vi "UnscentedKalmanFilter_SetXHat_Single.vi"(9 "xHat Value":dbl, 10 "Row":i32, 11 "in UnscentedKalmanFiilter":T1) -> (0 "Error":bool, 3 "out UnscentedKalmanFiilter":T1)   [LabVIEW 2019, in "Trajectory_Library.lvlib"]
doc: "Set an element of the initial state estimate x-hat.\n \nInputs:\n - inUnscentedKalmanFilter -- filter data cluster\n - row -- Row of x-hat.\n - value -- Value for element of x-hat.\n\nOutputs:\n - outUnscentedKalmanFilter -- updated filter data cluster\n - error -- If TRUE, an error occured."
uses:
  Trajectory_Library.lvlib
  <vilib>/Analysis/Matrix/Datatypes/RealMatrix.ctl
  <vilib>/Analysis/Matrix/NI_Matrix.lvlib
  TypeDef/MERWE_SCALED_SIGMA_PTS.ctl
  TypeDef/UNSCENTED_KALMAN_FILTER.ctl
  TypeDef/CALLBACK_FUNC_TYPE.ctl
panel:
  # "State Estimate <Statess,1>"
  # "<States, States>"
  # "<States, ?>"
  # "<Statess,  States>"
  # "<Outputs, Outputs>"
  # "<?, 1>"
  # "<?, 1>"
  # "State Estimate <Statess,1>"
  # "<States, States>"
  # "<States, ?>"
  # "<Statess,  States>"
  # "<Outputs, Outputs>"
  # "<?, 1>"
  # "<?, 1>"
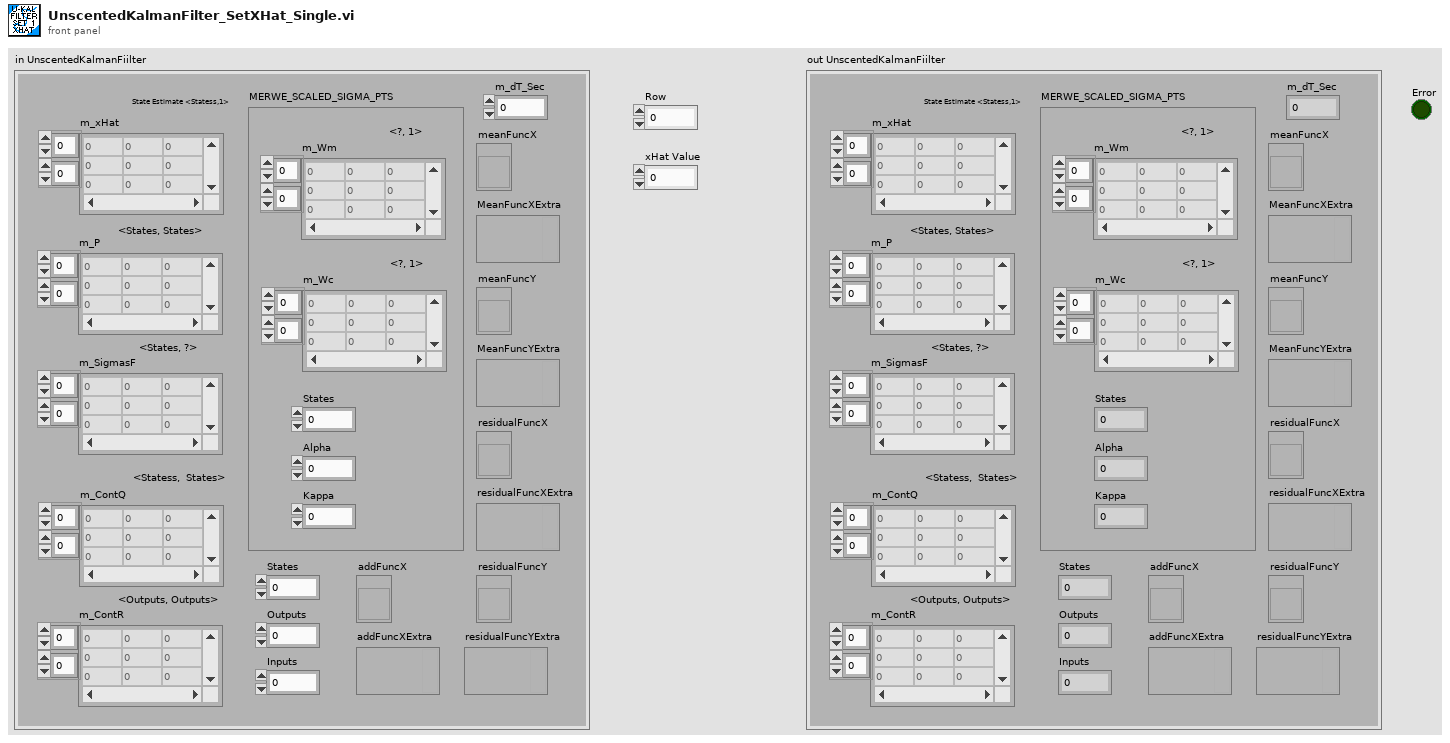
[diagram p1: front panel]
types:
  T1 = typedef "Trajectory_Library.lvlib/UNSCENTED_KALMAN_FILTER.ctl" = cluster{"m_P":T2, "m_xHat":T2, "States":i32, "Outputs":i32, "m_ContR":T2, "m_ContQ":T2, "m_SigmasF":T2, "m_dT_Sec":dbl, "MERWE_SCALED_SIGMA_PTS":T3, "meanFuncX":T4, "meanFuncY":T4, "residualFuncX":T4, "residualFuncY":T4, "addFuncX":T4, "addFuncXExtra":variant, "residualFuncYExtra":variant, "residualFuncXExtra":variant, "MeanFuncYExtra":variant, "MeanFuncXExtra":variant, "Inputs":i32}
  T2 = typedef "NI_Matrix.lvlib/RealMatrix.ctl" = dbl[][]
  T3 = typedef "Trajectory_Library.lvlib/MERWE_SCALED_SIGMA_PTS.ctl" = cluster{"m_Wm":T2, "States":i32, "Alpha":dbl, "m_Wc":T2, "Kappa":i32}
  T4 = typedef "Trajectory_Library.lvlib/CALLBACK_FUNC_TYPE.ctl" = refnum<vi>
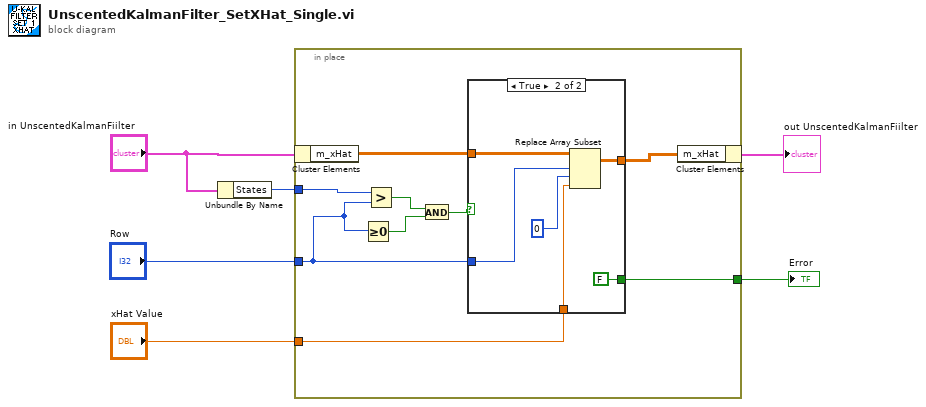
[diagram p0: block diagram]
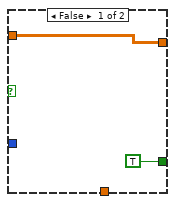
[diagram p2: hidden frame]
diagram:
  n1 = Unbundle By Name("in UnscentedKalmanFiilter") -> ("States"=w2:i32)
  n2 = in-place {
    in-place-border: "Row" -> [w9]
    in-place-border: "xHat Value" -> [w13]
    in-place-border: w2 -> [w10]
    in-place-border: [w7] -> w1
    n3 = in-place-cluster #1("in UnscentedKalmanFiilter") -> ("m_xHat"=w15:T2)
    n4 = Greater Or Equal To 0?(x=w9) -> (x >= 0?=w11:bool)
    n5 = Greater?(x=w10, y=w9) -> (0:w12:bool)
    n6 = And(x=w12, y=w11) -> (x .and. y?=w8:bool)
    n7 = case shown="True" w8 {
      tunnel: w15 -> [w17 w23]
      tunnel: [w17 w22] -> w14
      tunnel: w13 -> [_ w20]
      tunnel: w9 -> [_ w19]
      tunnel: [TRUE FALSE] -> w7
      frame False {
      }
      frame True {
        n8 = Replace Array Subset(array=w23, new element=w20, index (row)=w19, index (col)=0) -> (w22:T2)
      }
    }
    n9 = in-place-cluster #1("m_xHat"=w14) -> (→"out UnscentedKalmanFiilter":T1)
  }
  "Error" <- w1
